vi "Z Sample Stage Control.vi"(7 "Calling VI Ref":refnum<vi>) -> ()   [LabVIEW 2016]
uses:
  <vilib>/Utility/miscctls.llb/LVPointTypeDef.ctl
  Hardware Configuration/Hardware Configuration Controls/Device Type.ctl
  Hardware Configuration/Hardware Configuration Controls/Device Function.ctl
  Device Library/Stages/Stages Controls/Stage Actions.ctl
panel:
  in  "Down":bool
  in  "Up":bool
  in  "Position (µm)":dbl format="%#.3g"
  in  "Step Size (µm)":dbl=0.1
  in  "Quit":bool
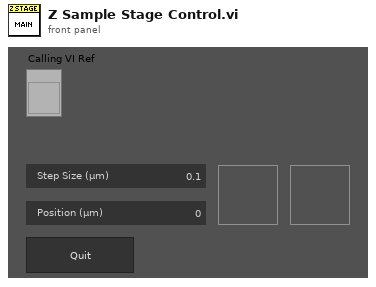
[diagram p1: front panel]
types:
  T1 = enum16{"Always On", "Always Off", "Off While Running"}
  T2 = typedef "LVPointTypeDef.ctl" = cluster{"Horizontal":i16, "Vertical":i16}
  T3 = typedef "Device Function.ctl" = enum16{"Primary", "Secondary", "Overview", "Wide Field Drift Correction", "642 nm Excitation", "560 nm Excitation", "546 nm Excitation", "488 nm Excitation", "405 nm Excitation", "Objective Drift Correction", "Objective XY", "Objective Z", "Sample XY", "Sample Coarse Z", "Sample Z", "4Pi Lower", "4Pi Upper", "Adj Cavity", "Line Scanning", "Alert"}
  T4 = typedef "Device Type.ctl" = enum16{"AOTF", "Camera", "Deformable Mirror", "Laser", "Shutter", "Stage", "Waveform", "Email"}
  T5 = typedef "Stage Actions.ctl" = enum16{"Get Position", "MVR", "MOVE", "HALT", "ONTARGET", "ERROR", "REFERENCE", "INIT", "VELOCITY", "STATUS", "EXIT", "HOME", "ZEROPOS", "NANOPOS", "ANALOG", "QUIT"}
  T6 = enum32{"Invalid", "Standard", "Closed", "Hidden", "Minimized", "Maximized"}
  T7 = typedef "LVRectTypeDef.ctl" = cluster{"Left":i16, "Top":i16, "Right":i16, "Bottom":i16}
  T8 = typedef "LVBoundsTypeDef.ctl" = cluster{"Width":u32, "Height":u32}
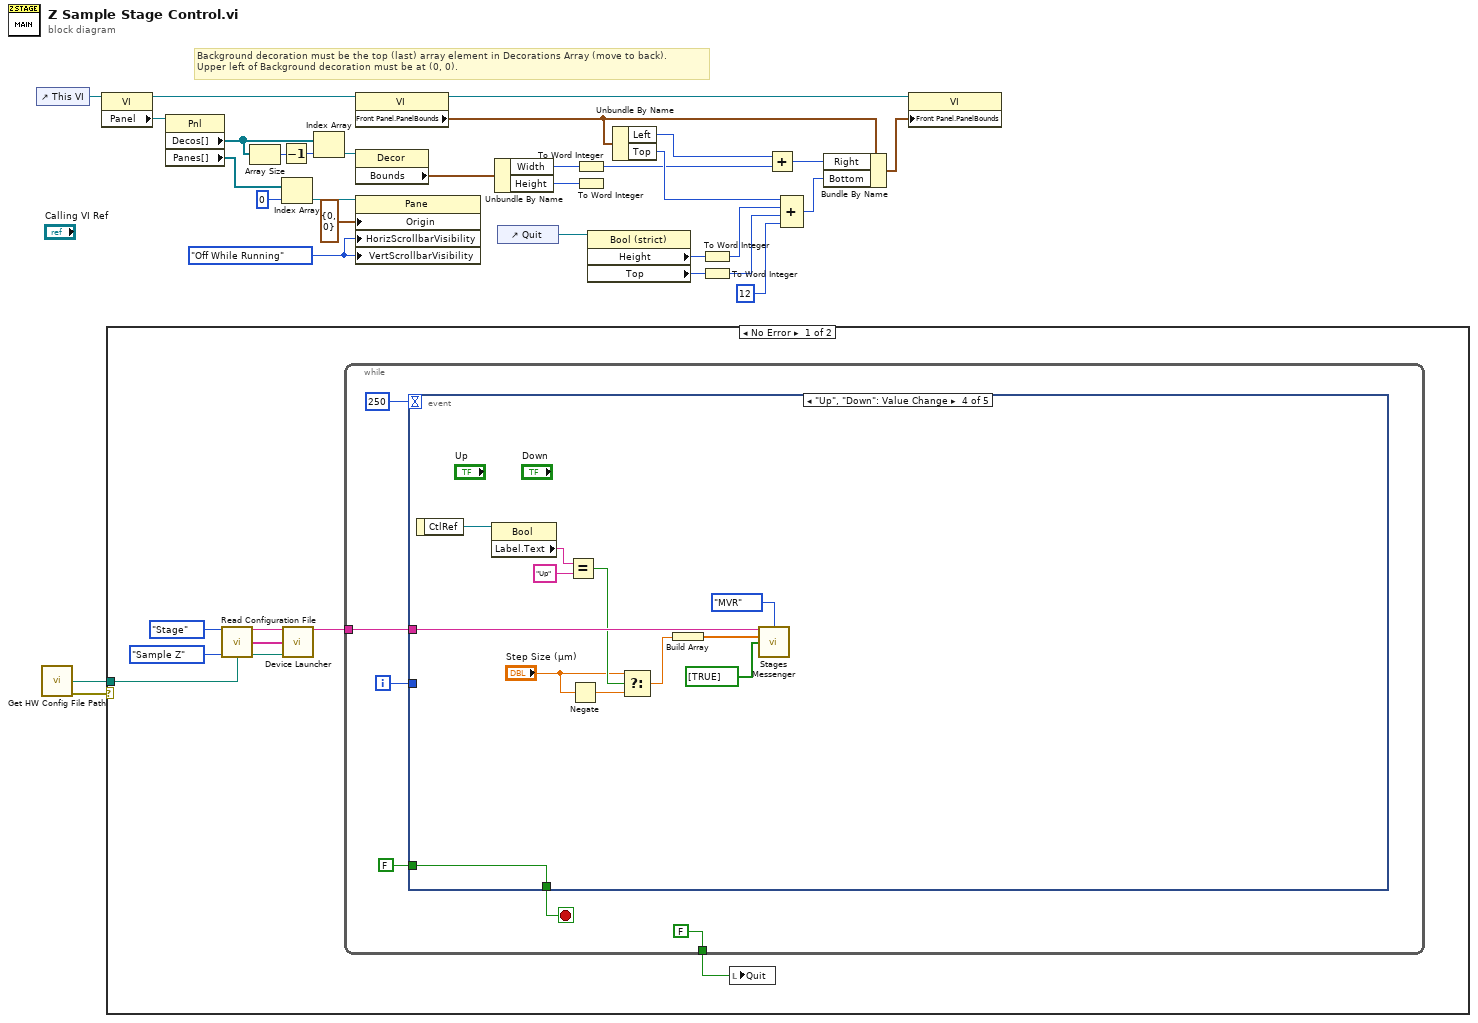
[diagram p0: block diagram]
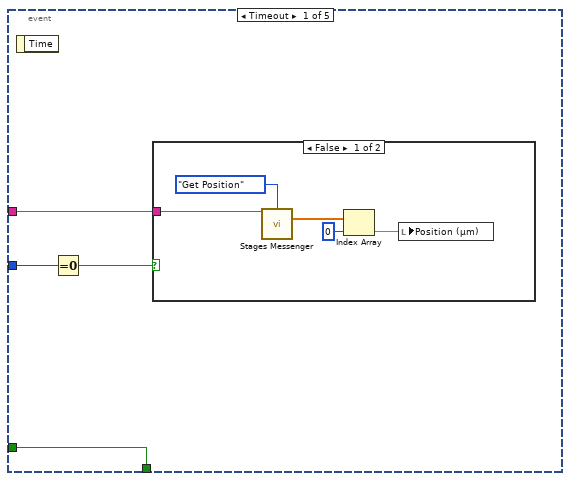
[diagram p2: hidden frame]
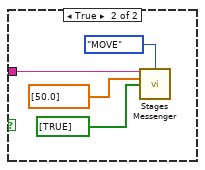
[diagram p3: hidden frame]
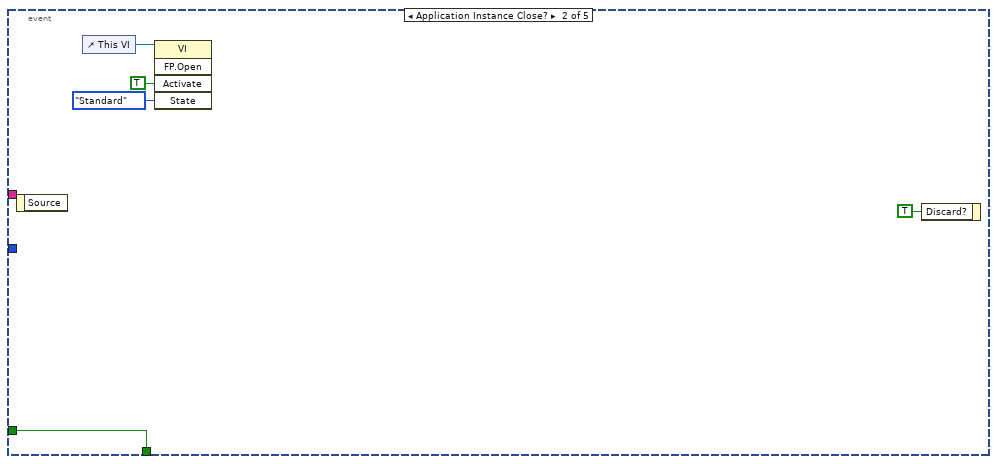
[diagram p4: hidden frame]
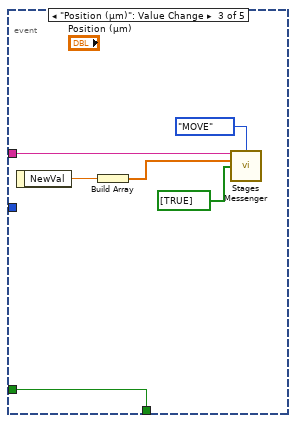
[diagram p5: hidden frame]
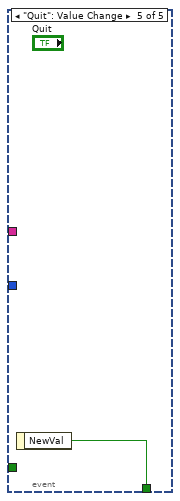
[diagram p6: hidden frame]
diagram:
  w12 = T1."Off While Running" ("Vertical Scrollbar Visibility")
  # "Background decoration must be the top (last) array element in Decorations Array (move to back).\nUpper left of Background decoration must be at (0, 0)."
  n1 = control-ref of="This VI"() -> (w4:refnum<vi>)
  n2 = call "Get HW Config File Path.vi"() -> ("File Path"=w30:path, "Error"=w31:errorcluster)  [unwired: 14 in]
  n3 = property class="VI"(reference=w4) -> (reference out=w13:refnum<vi>, "Panel"=w5:refnum<vi>)  [unwired: 1 in, 1 out]
  n4 = case shown="No Error" w31 {
    tunnel: w30 -> [w32 _]
    frame No Error {
      n5 = call "Read Configuration File.vi"("Device Type"=Device_Type."Stage", "Device Function"=Device_Function."Sample Z", "Config File Path"=w32) -> ("Unique Notifier Name"=w37:string, "Device Ports/IDs/Channels"=w39:string[], "Device Engine Path"=w38:path)  [unwired: 9 in, 1 out]
      n6 = call "Device Launcher.vi"("Notifier Name"=w37, "Device Ports/IDs/Channels"=w39, "Device Engine Path"=w38) -> ("Notifier Name"=w34:string)  [unwired: 11 in, 1 out]
      n7 = while {
        tunnel: w34 -> [w41]
        tunnel: [FALSE] -> w33
        i -> [w40]
        stop <- w43 stop-if-true
        n8 = event shown="[3] \"Up\", \"Down\": Value Change" {
          selector: _ -> [_ _ _ _ _]
          dyn-events: _ -> [_ _ _ _ _]
          timeout: 250 -> [_ _ _ _ _]
          tunnel: FALSE -> [w49 w62 w69 w81 _]
          tunnel: [w49 w62 w69 w81 w82] -> w43
          tunnel: w41 -> [w46 _ w66 w75 _]
          tunnel: w40 -> [w48 _ _ _ _]
          event Timeout {
            n9 = event-data() -> ()  [unwired: 1 in, 1 out]
            n10 = Equal To 0?(x=w48) -> (x = 0?=w47:bool)
            n11 = case shown="False" w47 {
              tunnel: w46 -> [w53 w57]
              frame False {
                n12 = call "Stages Messenger.vi"("Stage Notifier Name"=w53, "Actions"=Stage_Actions."Get Position") -> ("Positions"=w52:dbl[])  [unwired: 10 in, 3 out]
                n13 = Index Array(array=w52, index=0) -> (element=w50:dbl)
                n14 = local write "Position (µm)"(w50) -> ()
              }
              frame True {
                n15 = call "Stages Messenger.vi"("Stage Notifier Name"=w57, "Actions"=Stage_Actions."MOVE", "Setpoint"=dbl[] [50.0], "Axis"=bool[] [TRUE]) -> ()  [unwired: 8 in, 4 out]
              }
            }
          }
          event Application Instance Close? {
            n16 = event-data() -> ()  [unwired: 1 in, 1 out]
            n17 = control-ref of="This VI"() -> (w59:refnum<vi>)
            n18 = invoke class="VI" method="FP.Open"(reference=w59, "Activate"=TRUE ("Activate?"), "State"=T6."Standard") -> ()  [unwired: 2 in, 5 out]
            n19 = event-data("Discard?"=TRUE) -> ()  [unwired: 1 in, 1 out]
          }
          event "Position (µm)": Value Change {
            n20 = event-data() -> ("NewVal"=w68:dbl)  [unwired: 1 in]
            n21 = Build Array(w68) -> (w65:dbl[])
            n22 = call "Stages Messenger.vi"("Stage Notifier Name"=w66, "Actions"=Stage_Actions."MOVE", "Setpoint"=w65, "Axis"=bool[] [TRUE]) -> ()  [unwired: 8 in, 4 out]
          }
          event "Up", "Down": Value Change {
            n23 = event-data() -> ("CtlRef"=w80:refnum<vi>)  [unwired: 1 in]
            n24 = property class="Bool"(reference=w80) -> ("Label.Text"=w79:string)  [unwired: 1 in, 2 out]
            n25 = Equal?(x=w79, y="Up") -> (x = y?=w74:bool)
            n26 = Negate(x="Step Size (µm)") -> (-x=w72:dbl)
            n27 = Select(t="Step Size (µm)", s=w74, f=w72) -> (s? t:f=w71:dbl)
            n28 = Build Array(w71) -> (w70:dbl[])
            n29 = call "Stages Messenger.vi"("Stage Notifier Name"=w75, "Actions"=Stage_Actions."MVR", "Setpoint"=w70, "Axis"=bool[] [TRUE]) -> ()  [unwired: 8 in, 4 out]
          }
          event "Quit": Value Change {
            n30 = event-data() -> ("NewVal"=w82:bool)  [unwired: 1 in]
          }
        }
      }
      n31 = local write "Quit"(w33) -> ()
    }
    frame Error {
    }
  }
  n32 = property class="Pnl"(reference=w5) -> ("Decos[]"=w3:refnum<vi>[], "Panes[]"=w9:refnum<vi>[])  [unwired: 1 in, 2 out]
  n33 = Array Size(array=w3) -> (size(s)=w1:i32)
  n34 = Decrement(x=w1) -> (x-1=w2:i32)
  n35 = Index Array(array=w9, index=0) -> (element=w8:refnum<vi>)
  n36 = Index Array(array=w3, index=w2) -> (element=w11:refnum<vi>)
  n37 = property class="VI"(reference=w13) -> (reference out=w15:refnum<vi>, "Front Panel.PanelBounds"=w16:T7)  [unwired: 1 in, 1 out]
  n38 = property class="Decor"(reference=w11) -> ("Bounds"=w14:T8)  [unwired: 1 in, 2 out]
  n39 = property class="Pane"(reference=w8, "Origin"=T2 {"Horizontal"=0, "Vertical"=0}, "HorizScrollbarVisibility"=w12, "VertScrollbarVisibility"=w12) -> ()  [unwired: 1 in, 2 out]
  n40 = Unbundle By Name(w14) -> ("Width"=w19:u32, "Height"=w22:u32)
  n41 = control-ref of="Quit"() -> (w6:refnum<vi>)
  n42 = To Word Integer(number=w19) -> (16bit integer=w21:i16)
  n43 = To Word Integer(number=w22) -> ()  [unwired: 1 out]
  n44 = property class="Bool (strict)"(reference=w6) -> ("Height"=w24:u32, "Top"=w25:i32)  [unwired: 1 in, 2 out]
  n45 = Unbundle By Name(w16) -> ("Left"=w18:i16, "Top"=w29:i16)
  n46 = To Word Integer(number=w24) -> (16bit integer=w27:i16)
  n47 = To Word Integer(number=w25) -> (16bit integer=w28:i16)
  n48 = Add(x=w18, y=w21) -> (x+y=w20:i16)
  n49 = Compound Arithmetic op=ADD(w29, w27, w28, i16 12 ("y")) -> (w23:i16)
  n50 = Bundle By Name(cluster=w16, "Right"=w20, "Bottom"=w23) -> (w17:T7)
  n51 = property class="VI"(reference=w15, "Front Panel.PanelBounds"=w17) -> ()  [unwired: 1 in, 2 out]
